vi "SPI Close.vi"(8 "error in (no error)":errorcluster, 11 "SPI Device":T1) -> (0 "error out":errorcluster)   [LabVIEW 2020, in "wiringPi.lvlib"]
doc: "<b>_______________________________________________________________</b>\n** Author: Juan José Villacorta\n** LabVIEW wrapper for C library <b> wiringPi </b>,\n** https://github.com/WiringPi/WiringPi\n<b>_______________________________________________________________</b>\n/*\n * Close a SPI Device\n**********************************************************************************\n*/"
uses:
  wiringPi.lvlib
  Type Defs/SPI Dev.ctl
  Type Defs/SPI Channel.ctl
  Type Defs/SPI Device.ctl
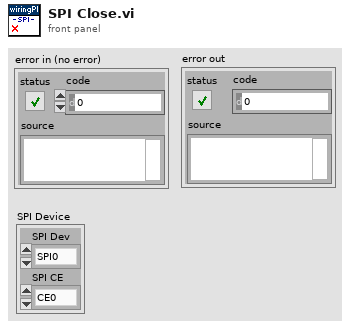
[diagram p1: front panel]
types:
  T1 = typedef "wiringPi.lvlib/SPI Device.ctl" = cluster{"SPI Dev":T2, "SPI CE":T3}
  T2 = typedef "wiringPi.lvlib/SPI Dev.ctl" = enum32{"SPI0", "SPI1"}
  T3 = typedef "wiringPi.lvlib/SPI Channel.ctl" = enum32{"CE0", "CE1", "CE2"}
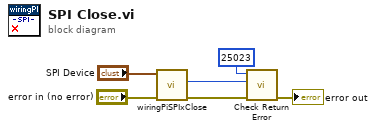
[diagram p0: block diagram]
diagram:
  n1 = call "wiringPiSPIxClose.vi"("error in (no error)"="error in (no error)", "SPI Device"="SPI Device") -> ("error out"=w3:errorcluster, "return"=w1:i32)  [unwired: 7 in, 1 out]
  n2 = call "Check Return Error.vi"("error in (no error)"=w3, "Return code"=w1, "Error number"=25023) -> ("error out"=→"error out":errorcluster)  [unwired: 8 in]
